vi "RDB Clear.vi"(8 "error in (no error)":errorcluster, 10 "RDB References":T4, 11 "Settings":T1={"UDP Receiver"=refnum, "UDP Sender"=refnum, "Valid Packet"=FALSE, "TCP"=refnum, "Network Settings"={"IP adress"="127.0.0.1", "RDB"={"Protocol"=enum."UDP", "Tx Port"=48270, "Rx Port"=10, "Buffer Size"=204800, "Timeout"=10}, "SCP"={"Protocol"=enum."TCP", "Tx Port"=48191, "Rx Port"=48191, "Buffer Size"=204800, "Timeout"=10}}, "vclient"=path "", "paeseHandle"=0, "builderHandle"=0}) -> (0 "error out":errorcluster)   [LabVIEW 2023, in "RDB.lvlib"]
uses:
  RDB.lvlib
  RDB References.ctl
  DataContainer/DataContainer.lvclass
  Engine/Type/Settings.ctl
  Shared/Network Settings.ctl
  Shared/Protocol.ctl
  Shared/Vires VTD Shared.lvlib
  Engine/Vires VTD Engine.lvlib
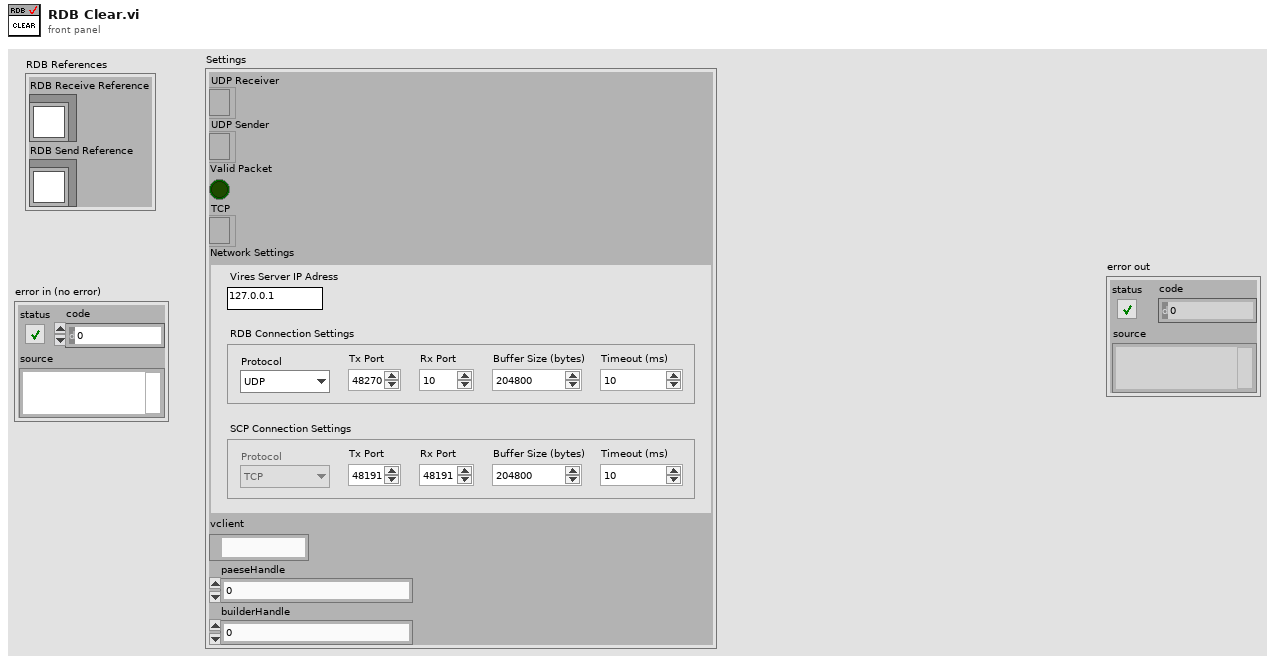
[diagram p1: front panel]
types:
  T1 = typedef "Vires VTD Engine.lvlib/Settings.ctl" = cluster{"UDP Receiver":refnum<k16>, "UDP Sender":refnum<k16>, "Valid Packet":bool, "TCP":refnum<k5>, "Network Settings":T2, "vclient":path, "paeseHandle":u64, "builderHandle":u64}
  T2 = typedef "Vires VTD Shared.lvlib/Network Settings.ctl" = cluster{"IP adress":string, "RDB":cluster{"Protocol":T3, "Tx Port":u16, "Rx Port":u16, "Buffer Size":i32, "Timeout":u16}, "SCP":cluster{"Protocol":T3, "Tx Port":u16, "Rx Port":u16, "Buffer Size":i32, "Timeout":u16}}
  T3 = typedef "Vires VTD Shared.lvlib/Protocol.ctl" = enum16{"UDP", "TCP"}
  T4 = typedef "RDB.lvlib/RDB References.ctl" = cluster{"RDB Receive Reference":refnum<class "DataContainer.lvclass">, "RDB Send Reference":refnum<class "DataContainer.lvclass">}
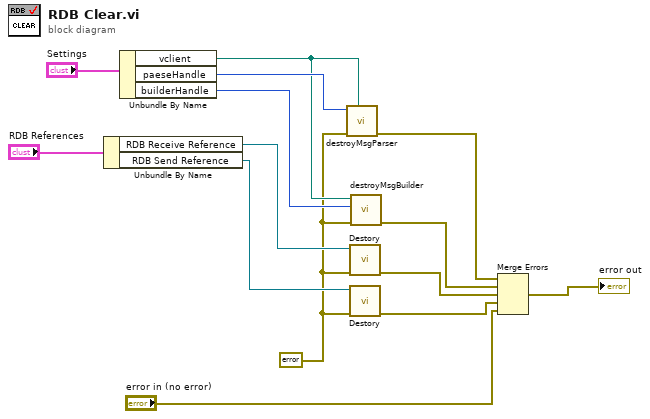
[diagram p0: block diagram]
diagram:
  w1 = errorcluster {"status"=FALSE, "code"=0, "source"=""} ("error in (no error)")
  n1 = Unbundle By Name("RDB References") -> ("RDB Receive Reference"=w6:refnum<class "DataContainer.lvclass">, "RDB Send Reference"=w5:refnum<class "DataContainer.lvclass">)
  n2 = Unbundle By Name("Settings") -> ("vclient"=w11:path, "paeseHandle"=w12:u64, "builderHandle"=w10:u64)
  n3 = call "destroyMsgParser.vi"("path in"=w11, "error in (no error)"=w1, "parserHandle"=w12) -> ("error out"=w9:errorcluster)  [unwired: 8 in]
  n4 = call-dynamic "Destory.vi"("error in (no error)"=w1, "DataContainer in"=w6) -> ("error out"=w4:errorcluster)  [unwired: 8 in, 1 out]
  n5 = call-dynamic "Destory.vi"("error in (no error)"=w1, "DataContainer in"=w5) -> ("error out"=w3:errorcluster)  [unwired: 8 in, 1 out]
  n6 = call "destroyMsgBuilder.vi"("error in (no error)"=w1, "builderHandle"=w10, "path in"=w11) -> ("error out"=w8:errorcluster)  [unwired: 8 in]
  n7 = Merge Errors(w9, w8, w4, w3, "error in (no error)") -> (→"error out":errorcluster)
